vi "Populate Document Elements.vi"(8 "error in (no error)":errorcluster, 11 "xwpfDocument in":refnum<class "xwpfDocument.lvclass">) -> (0 "error out":errorcluster, 3 "xwpfDocument out":refnum<class "xwpfDocument.lvclass">)   [LabVIEW 2017, in "Word_Specific.lvlib" / "xwpfDocument.lvclass"]
uses:
  xwpfDocument.lvclass
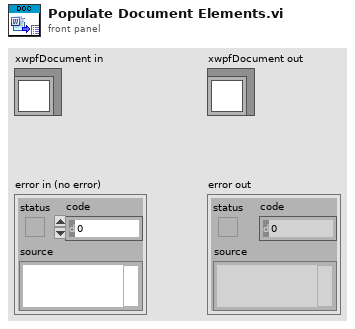
[diagram p1: front panel]
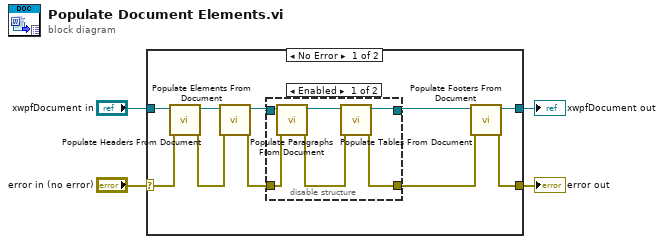
[diagram p0: block diagram]
diagram:
  n1 = case shown="No Error" "error in (no error)" {
    selector: "error in (no error)" -> [w13 w23]
    tunnel: [w11 w23] -> w3
    tunnel: [w12 w22] -> w1
    tunnel: "xwpfDocument in" -> [w14 w22]
    frame No Error {
      n2 = call "Populate Headers From Document.vi"("error in (no error)"=w13, "xwpfDocument in"=w14) -> ("error out"=w6:errorcluster, "xwpfDocument out"=w8:refnum<class "xwpfDocument.lvclass">)  [unwired: 8 in]
      n3 = call "Populate Elements From Document.vi"("error in (no error)"=w6, "xwpfDocument in"=w8) -> ("error out"=w5:errorcluster, "xwpfDocument out"=w7:refnum<class "xwpfDocument.lvclass">)  [unwired: 8 in]
      n4 = disable-structure shown="Enabled" {
        disable-tunnel: [w19 w21] -> w10
        disable-tunnel: [w17 _] -> w9
        disable-tunnel: w7 -> [w16 w21]
        disable-tunnel: w5 -> [w15 _]
        frame Enabled {
          n5 = call "Populate Paragraphs From Document.vi"("error in (no error)"=w15, "xwpfDocument in"=w16) -> ("error out"=w18:errorcluster, "xwpfDocument out"=w20:refnum<class "xwpfDocument.lvclass">)  [unwired: 8 in]
          n6 = call "Populate Tables From Document.vi"("error in (no error)"=w18, "xwpfDocument in"=w20) -> ("error out"=w17:errorcluster, "xwpfDocument out"=w19:refnum<class "xwpfDocument.lvclass">)  [unwired: 8 in]
        }
        frame Disabled {
        }
      }
      n7 = call "Populate Footers From Document.vi"("error in (no error)"=w9, "xwpfDocument in"=w10) -> ("error out"=w11:errorcluster, "xwpfDocument out"=w12:refnum<class "xwpfDocument.lvclass">)  [unwired: 8 in]
    }
    frame Error {
    }
  }
  "error out" <- w3
  "xwpfDocument out" <- w1
